vi "PLC_Xfer.vi"(8 "error in (no error)":errorcluster, 9 "RX Bytes":u32, 10 "TX":string, 11 "PLC Conn":refnum<visa-resource-name>) -> (0 "error out":errorcluster, 2 "RX":string, 3 "PLC Conn out":refnum<visa-resource-name>)   [LabVIEW 2018]
doc: "Use this template to build a VI to use as a subVI."
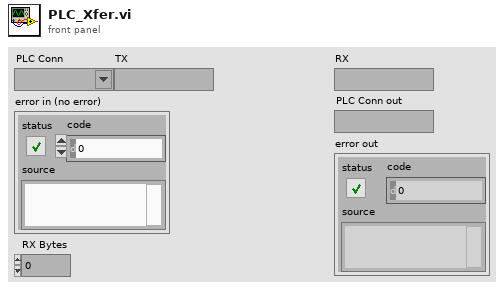
[diagram p1: front panel]
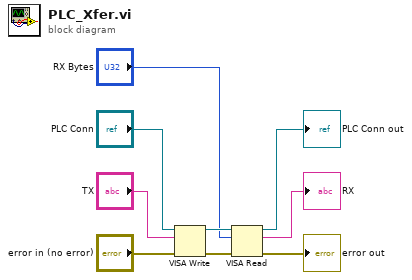
[diagram p0: block diagram]
diagram:
  n1 = VISA Write(VISA resource name="PLC Conn", write buffer="TX", error in (no error)="error in (no error)") -> (VISA resource name out=w8:refnum<visa-resource-name>, error out=w7:errorcluster)  [unwired: 1 out]
  n2 = VISA Read(VISA resource name=w8, byte count="RX Bytes", error in (no error)=w7) -> (VISA resource name out=→"PLC Conn out":refnum<visa-resource-name>, read buffer=→"RX":string, error out=→"error out":errorcluster)  [unwired: 1 out]
